vi "Add-size.vi"(11 "数组":string[][](array[string])) -> (3 "添加的数组":string[][](array[string]))   [LabVIEW 2025]
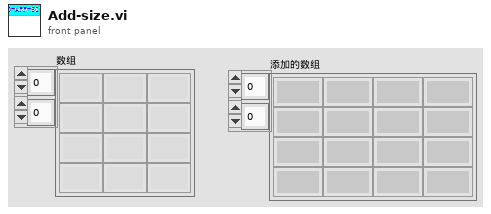
[diagram p1: front panel]
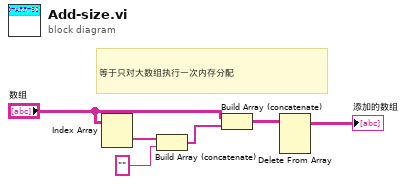
[diagram p0: block diagram]
diagram:
  # "等于只对大数组执行一次内存分配"
  n1 = Index Array(array="数组") -> (element=w6:string[])  [unwired: 2 in]
  n2 = Build Array (concatenate)(w6, "") -> (w4:string[])
  n3 = Build Array (concatenate)("数组", w4) -> (w2:string[][])
  n4 = Delete From Array(array=w2) -> (array with subset deleted=→"添加的数组":string[][])  [unwired: 3 in, 1 out]
